vi "D4xxx Set Values.vi"(7 "Function":enum16{"DCV", "ACV", "DCI", "ACI", "R", "WBV"}(ring), 8 "error in":errorcluster, 9 "Frequency":dbl, 10 "Value":dbl, 11 "4xxx":refnum<visa-resource-name>) -> (0 "error out":errorcluster, 3 "Session Out":refnum<visa-resource-name>)   [LabVIEW 2011]
doc: "Set value, frequency and function of Datron 4xxx series calibrators."
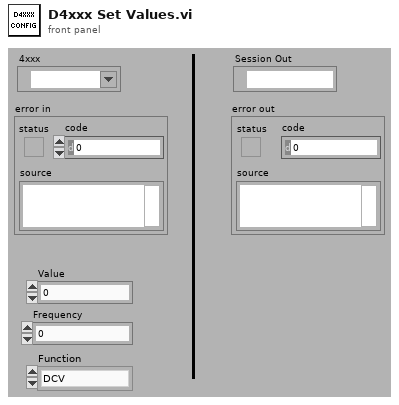
[diagram p1: front panel]
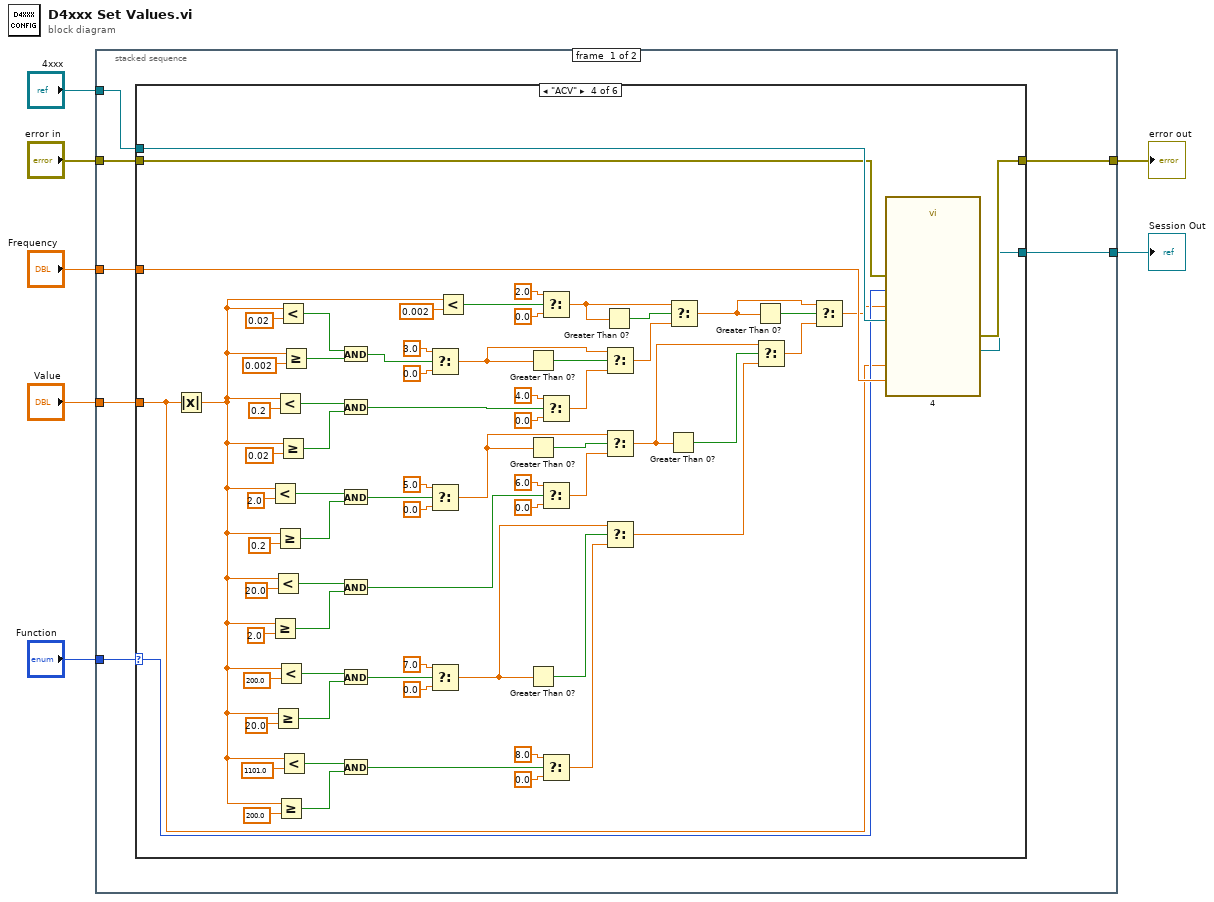
[diagram p0: block diagram]
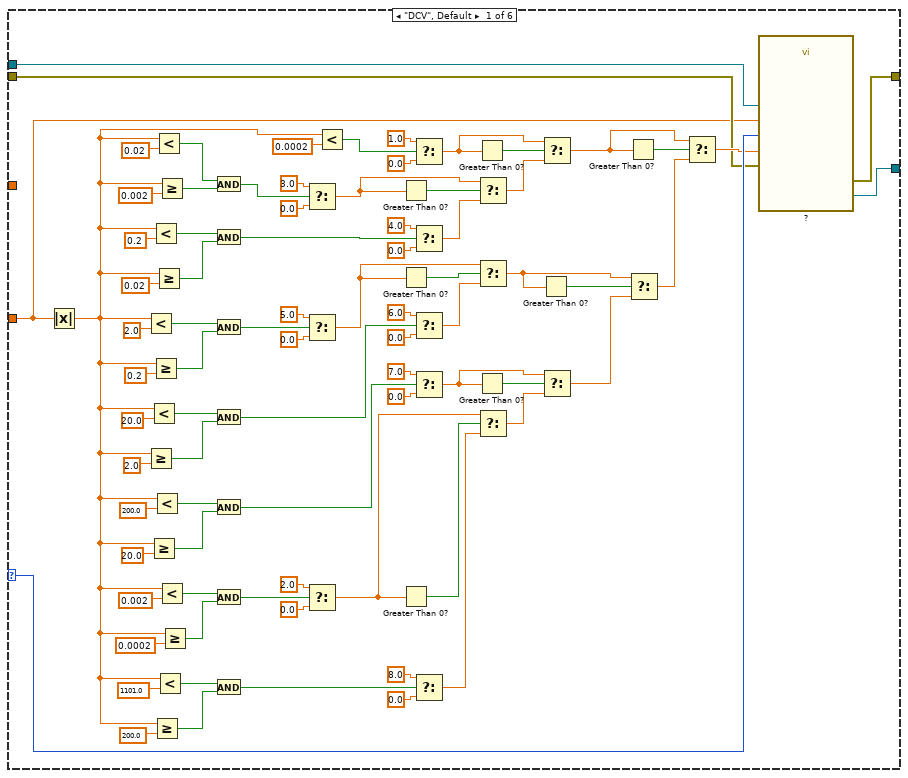
[diagram p2: hidden frame]
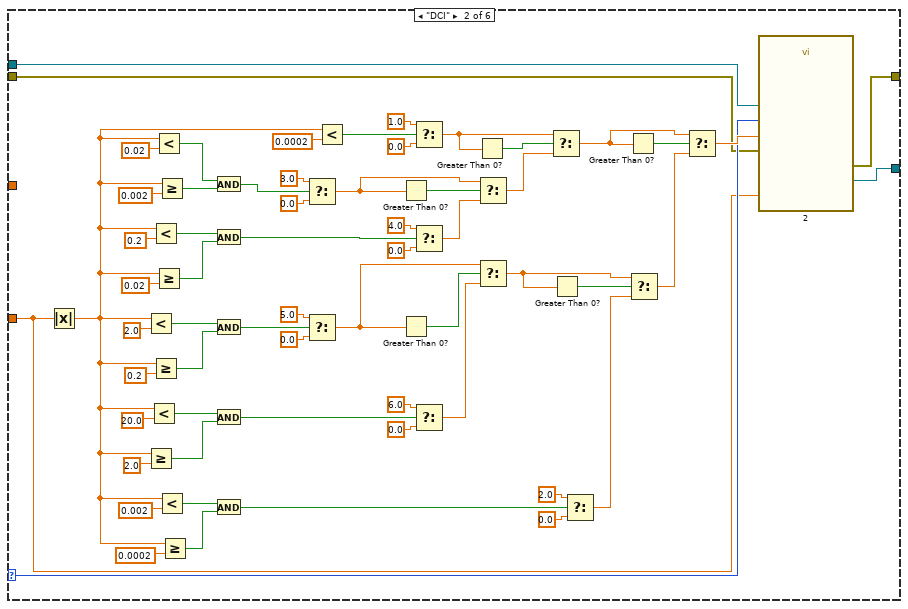
[diagram p3: hidden frame]
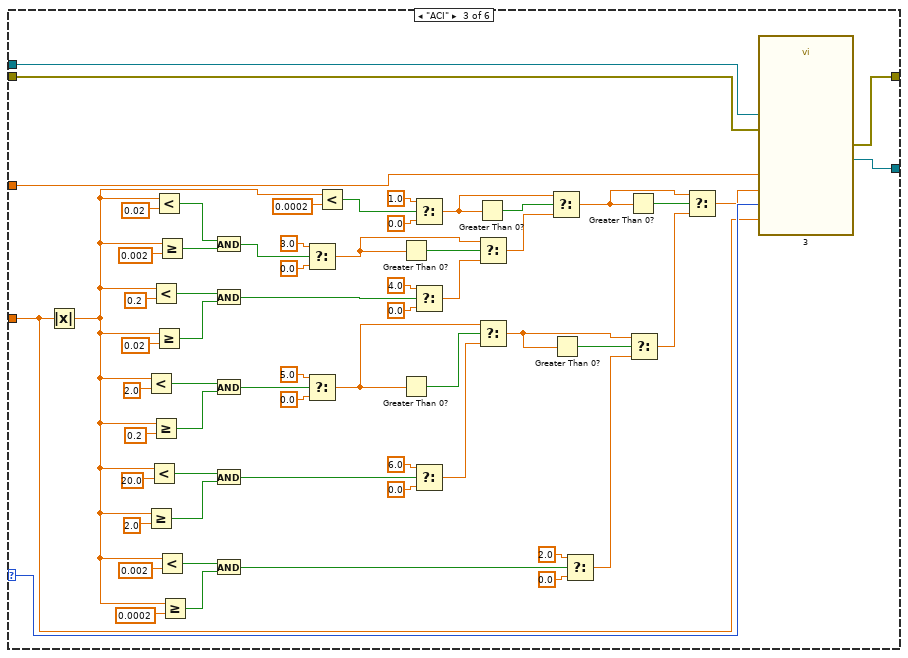
[diagram p4: hidden frame]
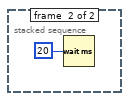
[diagram p7: hidden frame]
diagram:
  n1 = stacked-sequence {
    tunnel: "4xxx" -> [w14 _]
    tunnel: "Function" -> [w13 _]
    tunnel: "Value" -> [w12 _]
    tunnel: "Frequency" -> [w11 _]
    tunnel: [w10 _] -> w5
    tunnel: "error in" -> [w9 _]
    tunnel: [w8 _] -> w7
    frame #0 {
      n2 = case shown="\"ACV\"" w13 {
        selector: w13 -> [w32 w103 w166 w228 _ _]
        tunnel: w12 -> [w15 w97 w159 w222 _ _]
        tunnel: w14 -> [w33 w104 w167 w229 w296 w298]
        tunnel: w11 -> [_ _ w164 w230 _ _]
        tunnel: [w17 w100 w161 w224 w295 w297] -> w10
        tunnel: w9 -> [w18 w99 w162 w225 w295 w297]
        tunnel: [w16 w98 w160 w223 w296 w298] -> w8
        frame "DCV", Default {
          n3 = Absolute Value(x=w15) -> (abs(x)=w19:dbl)
          n4 = Less?(x=w19, y=2.0) -> (x < y?=w72:bool)
          n5 = Greater Or Equal?(x=w19, y=2.0) -> (x >= y?=w71:bool)
          n6 = Less?(x=w19, y=20.0) -> (x < y?=w65:bool)
          n7 = Greater Or Equal?(x=w19, y=20.0) -> (x >= y?=w64:bool)
          n8 = Less?(x=w19, y=0.2) -> (x < y?=w79:bool)
          n9 = Greater Or Equal?(x=w19, y=0.2) -> (x >= y?=w78:bool)
          n10 = Less?(x=w19, y=200.0) -> (x < y?=w58:bool)
          n11 = Greater Or Equal?(x=w19, y=200.0) -> (x >= y?=w57:bool)
          n12 = Less?(x=w19, y=0.02) -> (x < y?=w92:bool)
          n13 = Greater Or Equal?(x=w19, y=0.02) -> (x >= y?=w85:bool)
          n14 = Less?(x=w19, y=1101.0) -> (x < y?=w51:bool)
          n15 = Greater Or Equal?(x=w19, y=0.002) -> (x >= y?=w91:bool)
          n16 = Less?(x=w19, y=0.002) -> (x < y?=w25:bool)
          n17 = Greater Or Equal?(x=w19, y=0.0002) -> (x >= y?=w31:bool)
          n18 = And(x=w92, y=w91) -> (x .and. y?=w90:bool)
          n19 = And(x=w79, y=w85) -> (x .and. y?=w84:bool)
          n20 = And(x=w72, y=w78) -> (x .and. y?=w77:bool)
          n21 = And(x=w65, y=w71) -> (x .and. y?=w70:bool)
          n22 = And(x=w58, y=w64) -> (x .and. y?=w63:bool)
          n23 = And(x=w25, y=w31) -> (x .and. y?=w30:bool)
          n24 = And(x=w51, y=w57) -> (x .and. y?=w56:bool)
          n25 = Select(t=3.0, s=w90, f=0.0) -> (s? t:f=w47:dbl)
          n26 = Select(t=5.0, s=w77, f=0.0) -> (s? t:f=w45:dbl)
          n27 = Select(t=2.0, s=w30, f=0.0) -> (s? t:f=w23:dbl)
          n28 = Less?(x=w19, y=0.0002) -> (x < y?=w95:bool)
          n29 = Greater Than 0?(x=w47) -> (x > 0?=w48:bool)
          n30 = Greater Than 0?(x=w45) -> (x > 0?=w46:bool)
          n31 = Greater Than 0?(x=w23) -> (x > 0?=w24:bool)
          n32 = Select(t=1.0, s=w95, f=0.0) -> (s? t:f=w41:dbl)
          n33 = Select(t=4.0, s=w84, f=0.0) -> (s? t:f=w43:dbl)
          n34 = Select(t=6.0, s=w70, f=0.0) -> (s? t:f=w44:dbl)
          n35 = Select(t=7.0, s=w63, f=0.0) -> (s? t:f=w49:dbl)
          n36 = Select(t=8.0, s=w56, f=0.0) -> (s? t:f=w22:dbl)
          n37 = Greater Than 0?(x=w41) -> (x > 0?=w42:bool)
          n38 = Greater Than 0?(x=w49) -> (x > 0?=w50:bool)
          n39 = Select(t=w47, s=w48, f=w43) -> (s? t:f=w40:dbl)
          n40 = Select(t=w45, s=w46, f=w44) -> (s? t:f=w38:dbl)
          n41 = Select(t=w23, s=w24, f=w22) -> (s? t:f=w21:dbl)
          n42 = Greater Than 0?(x=w38) -> (x > 0?=w39:bool)
          n43 = Select(t=w41, s=w42, f=w40) -> (s? t:f=w35:dbl)
          n44 = Select(t=w49, s=w50, f=w21) -> (s? t:f=w37:dbl)
          n45 = Greater Than 0?(x=w35) -> (x > 0?=w36:bool)
          n46 = Select(t=w38, s=w39, f=w37) -> (s? t:f=w34:dbl)
          n47 = Select(t=w35, s=w36, f=w34) -> (s? t:f=w20:dbl)
          n48 = call "?"("Session In"=w33, "VOLT:V"=w15, "RANGE"=w20, "FUNC"=w32, "error in"=w18) -> ("Session Out"=w16:refnum<visa-resource-name>, "error out"=w17:errorcluster)  [unwired: 21 in]
        }
        frame "DCI" {
          n49 = Absolute Value(x=w97) -> (abs(x)=w101:dbl)
          n50 = Less?(x=w101, y=2.0) -> (x < y?=w134:bool)
          n51 = Greater Or Equal?(x=w101, y=2.0) -> (x >= y?=w133:bool)
          n52 = Less?(x=w101, y=20.0) -> (x < y?=w127:bool)
          n53 = Less?(x=w101, y=0.2) -> (x < y?=w141:bool)
          n54 = Greater Or Equal?(x=w101, y=0.2) -> (x >= y?=w140:bool)
          n55 = Less?(x=w101, y=0.02) -> (x < y?=w154:bool)
          n56 = Greater Or Equal?(x=w101, y=0.02) -> (x >= y?=w147:bool)
          n57 = Greater Or Equal?(x=w101, y=0.002) -> (x >= y?=w153:bool)
          n58 = Less?(x=w101, y=0.002) -> (x < y?=w106:bool)
          n59 = Greater Or Equal?(x=w101, y=0.0002) -> (x >= y?=w112:bool)
          n60 = And(x=w154, y=w153) -> (x .and. y?=w152:bool)
          n61 = And(x=w141, y=w147) -> (x .and. y?=w146:bool)
          n62 = And(x=w134, y=w140) -> (x .and. y?=w139:bool)
          n63 = And(x=w127, y=w133) -> (x .and. y?=w132:bool)
          n64 = And(x=w106, y=w112) -> (x .and. y?=w111:bool)
          n65 = Select(t=3.0, s=w152, f=0.0) -> (s? t:f=w125:dbl)
          n66 = Select(t=5.0, s=w139, f=0.0) -> (s? t:f=w123:dbl)
          n67 = Less?(x=w101, y=0.0002) -> (x < y?=w157:bool)
          n68 = Greater Than 0?(x=w125) -> (x > 0?=w126:bool)
          n69 = Greater Than 0?(x=w123) -> (x > 0?=w124:bool)
          n70 = Select(t=1.0, s=w157, f=0.0) -> (s? t:f=w119:dbl)
          n71 = Select(t=4.0, s=w146, f=0.0) -> (s? t:f=w121:dbl)
          n72 = Select(t=6.0, s=w132, f=0.0) -> (s? t:f=w122:dbl)
          n73 = Greater Than 0?(x=w119) -> (x > 0?=w120:bool)
          n74 = Select(t=w125, s=w126, f=w121) -> (s? t:f=w118:dbl)
          n75 = Select(t=w123, s=w124, f=w122) -> (s? t:f=w116:dbl)
          n76 = Select(t=w119, s=w120, f=w118) -> (s? t:f=w114:dbl)
          n77 = Greater Than 0?(x=w116) -> (x > 0?=w117:bool)
          n78 = Select(t=2.0, s=w111, f=0.0) -> (s? t:f=w102:dbl)
          n79 = Greater Than 0?(x=w114) -> (x > 0?=w115:bool)
          n80 = Select(t=w116, s=w117, f=w102) -> (s? t:f=w113:dbl)
          n81 = Select(t=w114, s=w115, f=w113) -> (s? t:f=w105:dbl)
          n82 = call "2"("Session In"=w104, "CURR:A"=w97, "RANGE"=w105, "FUNC"=w103, "error in"=w99) -> ("Session Out"=w98:refnum<visa-resource-name>, "error out"=w100:errorcluster)  [unwired: 21 in]
        }
        frame "ACI" {
          n83 = Absolute Value(x=w159) -> (abs(x)=w163:dbl)
          n84 = Less?(x=w163, y=2.0) -> (x < y?=w197:bool)
          n85 = Greater Or Equal?(x=w163, y=2.0) -> (x >= y?=w196:bool)
          n86 = Less?(x=w163, y=20.0) -> (x < y?=w190:bool)
          n87 = Less?(x=w163, y=0.2) -> (x < y?=w204:bool)
          n88 = Greater Or Equal?(x=w163, y=0.2) -> (x >= y?=w203:bool)
          n89 = Less?(x=w163, y=0.02) -> (x < y?=w217:bool)
          n90 = Greater Or Equal?(x=w163, y=0.02) -> (x >= y?=w210:bool)
          n91 = Greater Or Equal?(x=w163, y=0.002) -> (x >= y?=w216:bool)
          n92 = Less?(x=w163, y=0.002) -> (x < y?=w169:bool)
          n93 = Greater Or Equal?(x=w163, y=0.0002) -> (x >= y?=w175:bool)
          n94 = And(x=w217, y=w216) -> (x .and. y?=w215:bool)
          n95 = And(x=w204, y=w210) -> (x .and. y?=w209:bool)
          n96 = And(x=w197, y=w203) -> (x .and. y?=w202:bool)
          n97 = And(x=w190, y=w196) -> (x .and. y?=w195:bool)
          n98 = And(x=w169, y=w175) -> (x .and. y?=w174:bool)
          n99 = Select(t=3.0, s=w215, f=0.0) -> (s? t:f=w188:dbl)
          n100 = Select(t=5.0, s=w202, f=0.0) -> (s? t:f=w186:dbl)
          n101 = Less?(x=w163, y=0.0002) -> (x < y?=w220:bool)
          n102 = Greater Than 0?(x=w188) -> (x > 0?=w189:bool)
          n103 = Greater Than 0?(x=w186) -> (x > 0?=w187:bool)
          n104 = Select(t=1.0, s=w220, f=0.0) -> (s? t:f=w182:dbl)
          n105 = Select(t=4.0, s=w209, f=0.0) -> (s? t:f=w184:dbl)
          n106 = Select(t=6.0, s=w195, f=0.0) -> (s? t:f=w185:dbl)
          n107 = Greater Than 0?(x=w182) -> (x > 0?=w183:bool)
          n108 = Select(t=w188, s=w189, f=w184) -> (s? t:f=w181:dbl)
          n109 = Select(t=w186, s=w187, f=w185) -> (s? t:f=w179:dbl)
          n110 = Select(t=w182, s=w183, f=w181) -> (s? t:f=w177:dbl)
          n111 = Greater Than 0?(x=w179) -> (x > 0?=w180:bool)
          n112 = Select(t=2.0, s=w174, f=0.0) -> (s? t:f=w168:dbl)
          n113 = Greater Than 0?(x=w177) -> (x > 0?=w178:bool)
          n114 = Select(t=w179, s=w180, f=w168) -> (s? t:f=w176:dbl)
          n115 = Select(t=w177, s=w178, f=w176) -> (s? t:f=w165:dbl)
          n116 = call "3"("Session In"=w167, "CURR:A"=w159, "FREQ:HZ"=w164, "RANGE"=w165, "FUNC"=w166, "error in"=w162) -> ("Session Out"=w160:refnum<visa-resource-name>, "error out"=w161:errorcluster)  [unwired: 20 in]
        }
        frame "ACV" {
          n117 = Absolute Value(x=w222) -> (abs(x)=w226:dbl)
          n118 = Less?(x=w226, y=2.0) -> (x < y?=w270:bool)
          n119 = Greater Or Equal?(x=w226, y=2.0) -> (x >= y?=w269:bool)
          n120 = Less?(x=w226, y=20.0) -> (x < y?=w263:bool)
          n121 = Greater Or Equal?(x=w226, y=20.0) -> (x >= y?=w262:bool)
          n122 = Less?(x=w226, y=0.2) -> (x < y?=w277:bool)
          n123 = Greater Or Equal?(x=w226, y=0.2) -> (x >= y?=w276:bool)
          n124 = Less?(x=w226, y=200.0) -> (x < y?=w256:bool)
          n125 = Greater Or Equal?(x=w226, y=200.0) -> (x >= y?=w255:bool)
          n126 = Less?(x=w226, y=0.02) -> (x < y?=w290:bool)
          n127 = Greater Or Equal?(x=w226, y=0.02) -> (x >= y?=w283:bool)
          n128 = Less?(x=w226, y=1101.0) -> (x < y?=w249:bool)
          n129 = Greater Or Equal?(x=w226, y=0.002) -> (x >= y?=w289:bool)
          n130 = And(x=w290, y=w289) -> (x .and. y?=w288:bool)
          n131 = And(x=w277, y=w283) -> (x .and. y?=w282:bool)
          n132 = And(x=w270, y=w276) -> (x .and. y?=w275:bool)
          n133 = And(x=w263, y=w269) -> (x .and. y?=w268:bool)
          n134 = And(x=w256, y=w262) -> (x .and. y?=w261:bool)
          n135 = And(x=w249, y=w255) -> (x .and. y?=w254:bool)
          n136 = Select(t=3.0, s=w288, f=0.0) -> (s? t:f=w244:dbl)
          n137 = Select(t=5.0, s=w275, f=0.0) -> (s? t:f=w242:dbl)
          n138 = Select(t=7.0, s=w261, f=0.0) -> (s? t:f=w247:dbl)
          n139 = Less?(x=w226, y=0.002) -> (x < y?=w293:bool)
          n140 = Greater Than 0?(x=w244) -> (x > 0?=w245:bool)
          n141 = Greater Than 0?(x=w242) -> (x > 0?=w243:bool)
          n142 = Greater Than 0?(x=w247) -> (x > 0?=w248:bool)
          n143 = Select(t=2.0, s=w293, f=0.0) -> (s? t:f=w238:dbl)
          n144 = Select(t=4.0, s=w282, f=0.0) -> (s? t:f=w240:dbl)
          n145 = Select(t=6.0, s=w268, f=0.0) -> (s? t:f=w241:dbl)
          n146 = Select(t=8.0, s=w254, f=0.0) -> (s? t:f=w246:dbl)
          n147 = Greater Than 0?(x=w238) -> (x > 0?=w239:bool)
          n148 = Select(t=w244, s=w245, f=w240) -> (s? t:f=w237:dbl)
          n149 = Select(t=w242, s=w243, f=w241) -> (s? t:f=w235:dbl)
          n150 = Select(t=w247, s=w248, f=w246) -> (s? t:f=w234:dbl)
          n151 = Greater Than 0?(x=w235) -> (x > 0?=w236:bool)
          n152 = Select(t=w238, s=w239, f=w237) -> (s? t:f=w232:dbl)
          n153 = Greater Than 0?(x=w232) -> (x > 0?=w233:bool)
          n154 = Select(t=w235, s=w236, f=w234) -> (s? t:f=w231:dbl)
          n155 = Select(t=w232, s=w233, f=w231) -> (s? t:f=w227:dbl)
          n156 = call "4"("Session In"=w229, "RANGE"=w227, "FUNC"=w228, "VOLT_V"=w222, "FREQ_HZ"=w230, "error in"=w225) -> ("Session Out"=w223:refnum<visa-resource-name>, "error out"=w224:errorcluster)  [unwired: 20 in]
        }
        frame "R" {
          # "DODELAT!"
        }
        frame "WBV" {
          # "DODELAT!"
        }
      }
    }
    frame #1 {
      n157 = Wait (ms)(milliseconds to wait=u32 20 ("millisecond multiple")) -> ()  [unwired: 1 out]
    }
  }
  "Session Out" <- w7
  "error out" <- w5
